vi "Remove Empty Rows - subVI.vi"(11 "Distance [cm] | Voltage [V]":dbl[][](array[numeric])) -> (3 "Valid calibration points":dbl[][](array[numeric]))   [LabVIEW 2025]
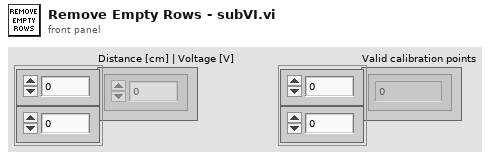
[diagram p1: front panel]
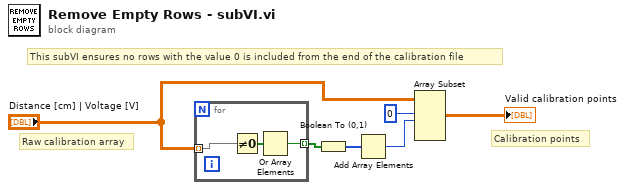
[diagram p0: block diagram]
diagram:
  # "Calibration points"
  # "Raw calibration array"
  # "This subVI ensures no rows with the value 0 is included from the end of the calibration file"
  n1 = for {
    tunnel: "Distance [cm] | Voltage [V]" -> [w9] mode=indexing
    tunnel: [w7] -> w1 mode=indexing
    n2 = Not Equal To 0?(x=w9) -> (x != 0?=w8:bool[])
    n3 = Or Array Elements(Boolean array=w8) -> (logical OR=w7:bool)
  }
  n4 = Boolean To (0,1)(Boolean=w1) -> (0, 1=w3:i16[])
  n5 = Add Array Elements(numeric array=w3) -> (sum=w2:i16)
  n6 = Array Subset(array="Distance [cm] | Voltage [V]", index (row)=0 ("index"), length (row)=w2) -> (→"Valid calibration points":dbl[][])  [unwired: 2 in]
